vi "Write Results CSV.vi"(0 "results folder path":path, 5 "sequence_id":string, 7 "Step Results":T1[](array[typedef]), 9 "overall verdict":string, 11 "error in":errorcluster) -> (4 "file path":path, 15 "error out":errorcluster)   [LabVIEW 2026]
doc: "Writes the step results as a CSV report to results folder path\\<sequence_id>_<YYYYMMDD_HHMMSS>.csv, creating the folder if needed (an existing folder is not an error). Content: a header row step_no,step_name,result,reason,measured,target,duration_ms, one row per Step Result and a final line OVERALL,<overall verdict>. An empty folder path returns error 7 and writes nothing; an incoming error skips the write. AF-free."
uses:
  Typedefs/Step Result.ctl
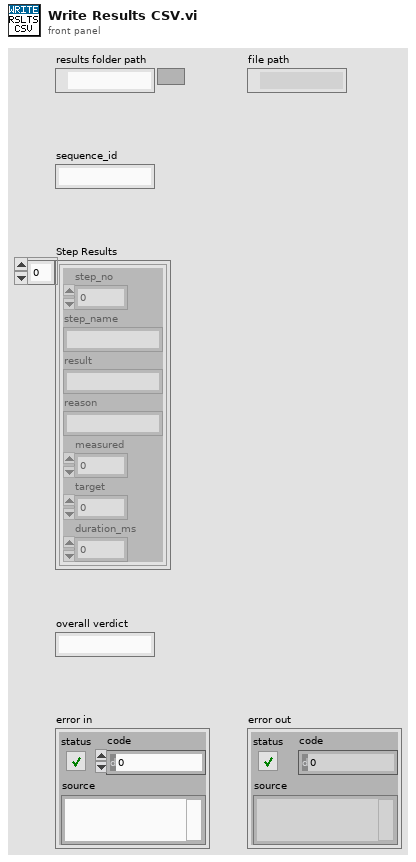
[diagram p1: front panel]
types:
  T1 = typedef "Step Result.ctl" = cluster{"step_no":i32, "step_name":string, "result":string, "reason":string, "measured":dbl, "target":dbl, "duration_ms":dbl}
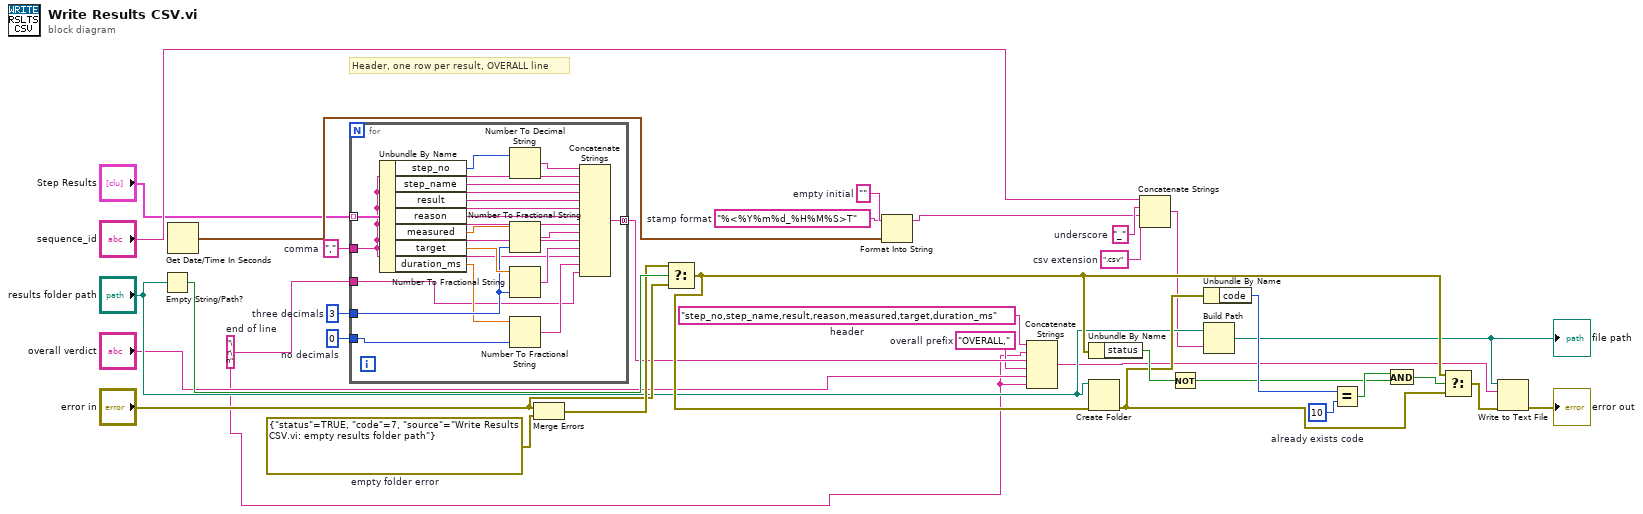
[diagram p0: block diagram]
diagram:
  w7 = "OVERALL,"  # overall prefix
  w9 = "step_no,step_name,result,reason,measured,target,duration_ms"  # header
  w10 = 0  # no decimals
  w11 = 3  # three decimals
  w5 = "\r\n"  # end of line
  w12 = ","  # comma
  w16 = ".csv"  # csv extension
  w18 = "_"  # underscore
  w22 = ""  # empty initial
  w20 = "%<%Y%m%d_%H%M%S>T"  # stamp format
  w29 = 10  # already exists code
  w34 = errorcluster {"status"=TRUE, "code"=7, "source"="Write Results CSV.vi: empty results folder path"}  # empty folder error
  # "Header, one row per result, OVERALL line"
  n1 = Empty String/Path?(string/path="results folder path") -> (empty?=w33:bool)
  n2 = Get Date/Time In Seconds() -> (seconds since 1Jan1904=w21:timestamp)
  n3 = for {
    tunnel: "Step Results" -> [w51] mode=indexing
    tunnel: w12 -> [w38]
    tunnel: w5 -> [w36]
    tunnel: w11 -> [w47]
    tunnel: w10 -> [w45]
    tunnel: [w35] -> w8 mode=concatenating
    n4 = Unbundle By Name(w51) -> ("step_no"=w50:i32, "step_name"=w43:string, "result"=w42:string, "reason"=w41:string, "measured"=w49:dbl, "target"=w48:dbl, "duration_ms"=w46:dbl)
    n5 = Number To Decimal String(number=w50) -> (decimal integer string=w44:string)  [unwired: 1 in]
    n6 = Number To Fractional String(number=w49, precision (6)=w47) -> (F-format string=w40:string)  [unwired: 2 in]
    n7 = Number To Fractional String(number=w48, precision (6)=w47) -> (F-format string=w39:string)  [unwired: 2 in]
    n8 = Number To Fractional String(number=w46, precision (6)=w45) -> (F-format string=w37:string)  [unwired: 2 in]
    n9 = Concatenate Strings(w44, w38, w43, w38, w42, w38, w41, w38, w40, w38, w39, w38, w37, w36) -> (w35:string)
  }
  n10 = Merge Errors("error in", w34) -> (w32:errorcluster)
  n11 = Select(t=w32, s=w33, f="error in") -> (s? t:f=w24:errorcluster)
  n12 = Format Into String(format string=w20, initial string=w22, w21) -> (resulting string=w17:string)  [unwired: 1 in, 1 out]
  n13 = Concatenate Strings(w9, w5, w8, w7, "overall verdict", w5) -> (w4:string)
  n14 = Unbundle By Name(w24) -> ("status"=w28:bool)
  n15 = Create Folder(path (use dialog)="results folder path", error in=w24) -> (error out=w23:errorcluster)  [unwired: 1 in, 2 out]
  n16 = Concatenate Strings("sequence_id", w18, w17, w16) -> (w14:string)
  n17 = Not(x=w28) -> (.not. x?=w26:bool)
  n18 = Unbundle By Name(w23) -> ("code"=w30:i32)
  n19 = Build Path(base path="results folder path", name or relative path=w14) -> (appended path=w2:path)
  "file path" <- w2
  n20 = Equal?(x=w30, y=w29) -> (x = y?=w27:bool)
  n21 = And(x=w27, y=w26) -> (x .and. y?=w25:bool)
  n22 = Select(t=w24, s=w25, f=w23) -> (s? t:f=w3:errorcluster)
  n23 = Write to Text File(file (use dialog)=w2, text=w4, error in=w3) -> (error out=→"error out":errorcluster)  [unwired: 1 in, 2 out]
